vi "Write TIFF.vi"(8 "error in (no error)":errorcluster, 10 "Path":path, 11 "ImageHandler:DT-ImageHandler in":refnum<class "DT-ImageHandler.lvclass">) -> (0 "error out":errorcluster, 3 "ImageHandler:DT-ImageHandler out":refnum<class "DT-ImageHandler.lvclass">)   [LabVIEW 2022 SP3, in "ImageHandler.lvlib" / "DT-ImageHandler.lvclass"]
uses:
  DT-ImageHandler.lvclass
  DT-ImageHandler.lvclass/DT-ImageHandler.ctl
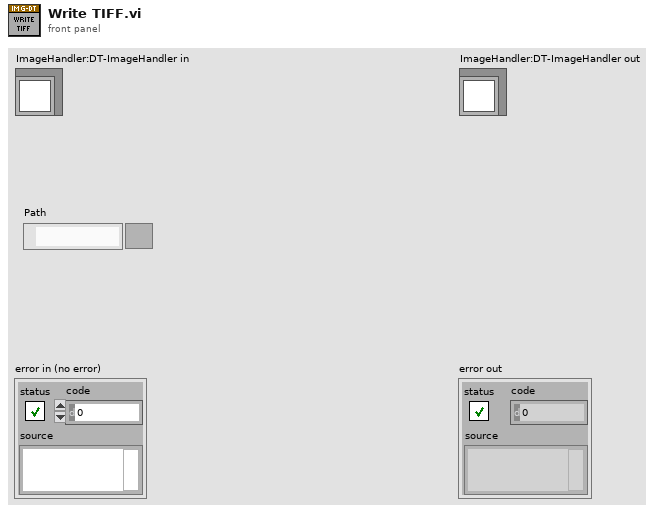
[diagram p1: front panel]
types:
  T1 = typedef "IMAQ Image.ctl" = refnum<image>
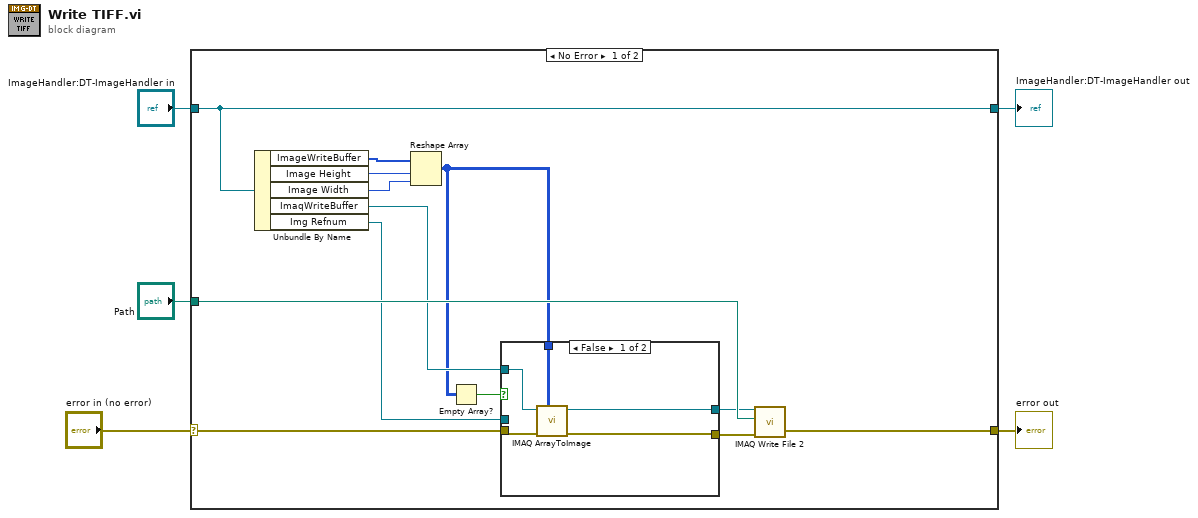
[diagram p0: block diagram]
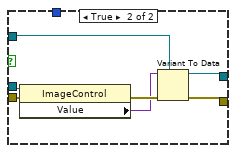
[diagram p2: hidden frame]
diagram:
  n1 = case shown="No Error" "error in (no error)" {
    selector: "error in (no error)" -> [w18 w32]
    tunnel: [w17 w32] -> w4
    tunnel: [w9 w31] -> w2
    tunnel: "ImageHandler:DT-ImageHandler in" -> [w9 w31]
    tunnel: "Path" -> [w16 _]
    frame No Error {
      n2 = Unbundle By Name(w9) -> ("ImageWriteBuffer"=w12:u16[], "Image Height"=w13:i32, "Image Width"=w14:i32, "ImaqWriteBuffer"=w11:T1, "Img Refnum"=w6:refnum<vi>)
      n3 = Reshape Array(w12, w13, w14) -> (w8:u16[][])
      n4 = Empty Array?(array=w8) -> (empty?=w7:bool)
      n5 = case shown="False" w7 {
        tunnel: w18 -> [w23 w30]
        tunnel: [w22 w27] -> w15
        tunnel: w11 -> [w21 w25]
        tunnel: [w20 w24] -> w10
        tunnel: w8 -> [w19 _]
        tunnel: w6 -> [_ w28]
        frame False {
          n6 = call "IMAQ ArrayToImage"("Image Pixels (U16)"=w19, "error in (no error)"=w23, "Image"=w21) -> ("error out"=w22:errorcluster, "Image Out"=w20:T1)  [unwired: 7 in]
        }
        frame True {
          n7 = property class="ImageControl"(reference=w28, error in=w30) -> (error out=w29:errorcluster, "Value"=w26:variant)  [unwired: 1 out]
          n8 = Variant To Data(error in=w29, type=w25, Variant=w26) -> (data=w24:T1, error out=w27:errorcluster)
        }
      }
      n9 = call-poly "IMAQ Write File 2"("error in (no error)"=w15, "File Path"=w16, "Image"=w10) -> ("error out"=w17:errorcluster)  [unwired: 7 in, 1 out]
    }
    frame Error {
    }
  }
  "error out" <- w4
  "ImageHandler:DT-ImageHandler out" <- w2
